vi "query Reference Level.vi"(8 "error in (no error)":errorcluster, 11 "Keysight 9020A in":refnum<class "Keysight 9020A.lvclass">) -> (0 "error out":errorcluster, 2 "Ref Level":dbl, 3 "Keysight 9020A out":refnum<class "Keysight 9020A.lvclass">)   [LabVIEW 2023, in "Spectrum Analyzer.lvlib" / "Keysight 9020A.lvclass"]
uses:
  Keysight 9020A.lvclass
  Keysight 9020A.lvclass/Keysight 9020A.ctl
  Spectrum Analyzer.lvlib
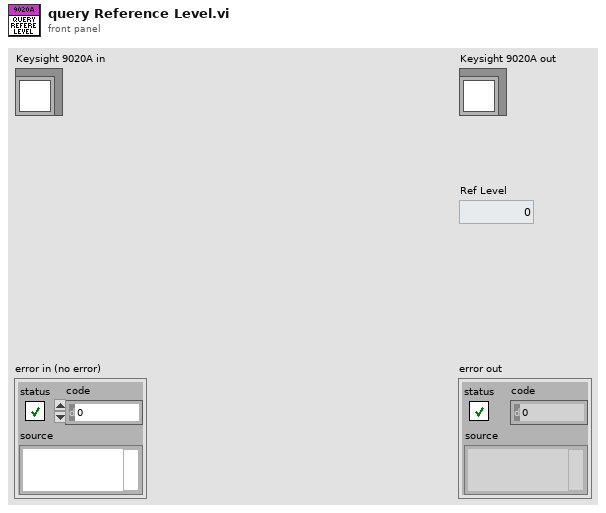
[diagram p1: front panel]
types:
  T1 = typedef "Spectrum Analyzer.lvlib/TYPE Measurement Preset.ctl" = enum16{"Sweep SA Mode", "Channel Power", "Occupied BW", "ACP", "Spurious Emission", "Spurious Emission Mask", "Burst Power (Transmit Power)"}
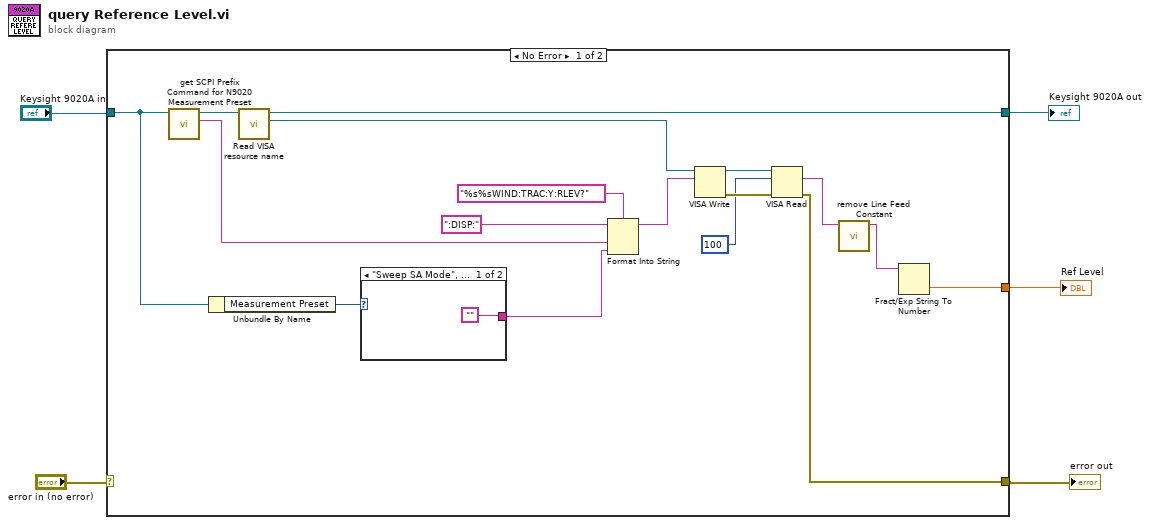
[diagram p0: block diagram]
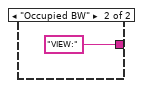
[diagram p2: hidden frame]
diagram:
  n1 = case shown="No Error" "error in (no error)" {
    selector: "error in (no error)" -> [_ w25]
    tunnel: "Keysight 9020A in" -> [w8 w26]
    tunnel: [w22 w26] -> w4
    tunnel: [w10 w25] -> w2
    tunnel: [w9 _] -> w1
    frame No Error {
      n2 = call "get SCPI Prefix Command for N9020 Measurement Preset.vi"("Keysight 9020A in"=w8) -> ("SCPI Prefix Command"=w16:string, "Keysight 9020A out"=w17:refnum<class "Keysight 9020A.lvclass">)  [unwired: 8 in, 1 out]
      n3 = Unbundle By Name(w8) -> ("Measurement Preset"=w7:T1)
      n4 = call "Read VISA resource name.vi"("Keysight 9020A in"=w17) -> ("VISA resource name"=w19:refnum<visa-resource-name>, "Keysight 9020A out"=w22:refnum<class "Keysight 9020A.lvclass">)  [unwired: 8 in, 1 out]
      n5 = case shown="\"Sweep SA Mode\", Default" w7 {
        tunnel: ["" "VIEW:"] -> w6
        frame "Sweep SA Mode", Default {
        }
        frame "Occupied BW" {
        }
      }
      n6 = Format Into String(format string="%s%sWIND:TRAC:Y:RLEV?", initial string=":DISP:", w16, w6) -> (resulting string=w18:string)  [unwired: 1 in, 1 out]
      n7 = VISA Write(VISA resource name=w19, write buffer=w18) -> (VISA resource name out=w15:refnum<visa-resource-name>, error out=w14:errorcluster)  [unwired: 1 in, 1 out]
      n8 = VISA Read(VISA resource name=w15, byte count=u32 100, error in (no error)=w14) -> (read buffer=w12:string, error out=w10:errorcluster)  [unwired: 2 out]
      n9 = call "remove Line Feed Constant.vi"("Input String"=w12) -> ("Line Feed Removed String"=w11:string)  [unwired: 10 in]
      n10 = Fract/Exp String To Number(string=w11) -> (number=w9:dbl)  [unwired: 3 in, 1 out]
    }
    frame Error {
    }
  }
  "error out" <- w2
  "Keysight 9020A out" <- w4
  "Ref Level" <- w1
